vi "Configure Reporting Dialog.vi"(8 "error in (no error)":errorcluster, 11 "Execution UI In":refnum<class "Execution UI.lvclass">) -> (0 "error out":errorcluster, 2 "Reporting Enabled?":bool, 3 "Execution UI Out":refnum<class "Execution UI.lvclass">)   [LabVIEW 2020, in "Execution UI.lvclass"]
uses:
  Execution UI.lvclass
  Framework/Report Plugin/Report Plugin.lvclass
  Framework/Plugin Loader/Plugin Loader.lvlib
  Configuration Manager/UI Configuration Manager.lvclass
  Framework/Configuration Manager/Configuration Manager.lvclass
  Framework/Plugin/Plugin.lvclass
panel:
  in  "Reports Plugins":i32(listbox)
  in  "Configure":bool
  in  "Commit":bool
  in  "Cancel":bool
  # "Double Click to toggle active plugin"
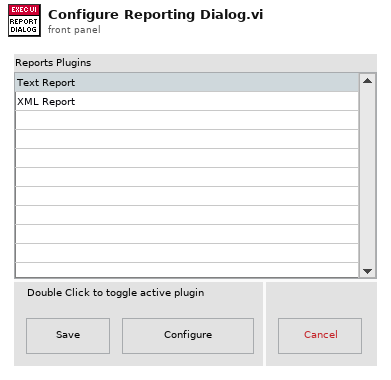
[diagram p1: front panel]
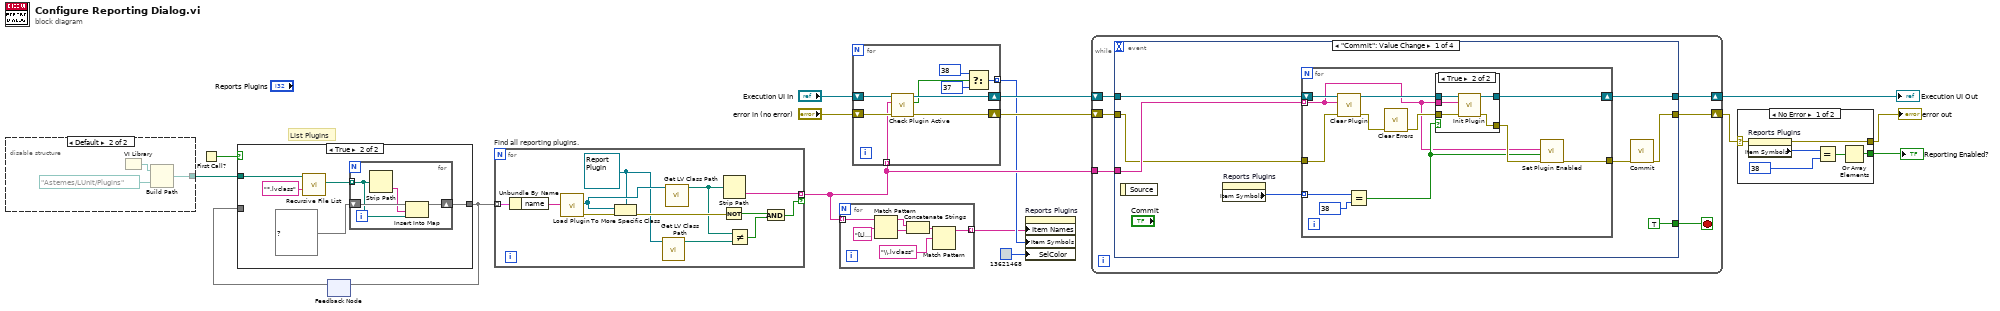
[diagram p0: block diagram]
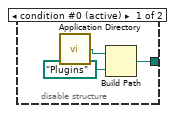
[diagram p2: hidden frame]
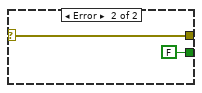
[diagram p4: hidden frame]
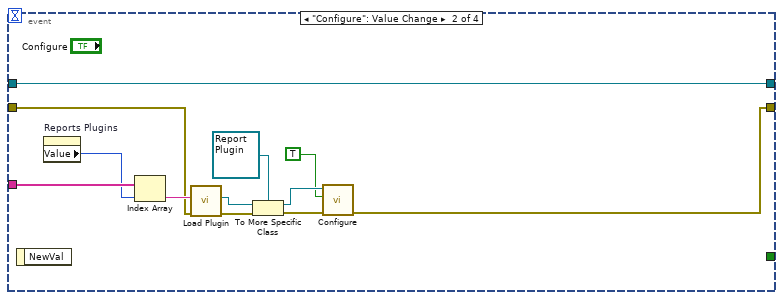
[diagram p6: hidden frame]
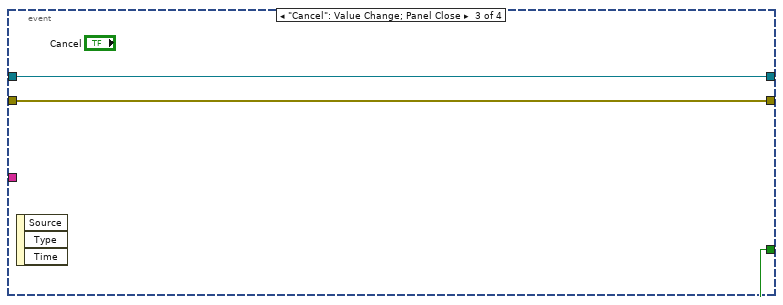
[diagram p7: hidden frame]
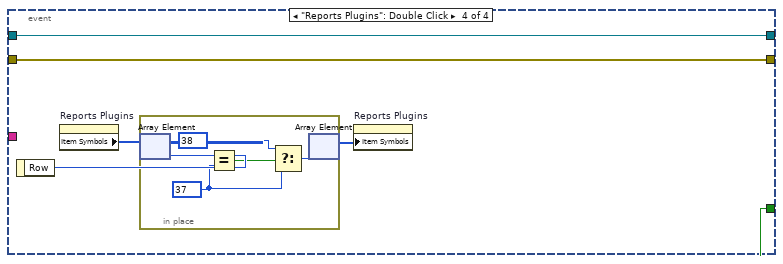
[diagram p8: hidden frame]
diagram:
  # "List Plugins"
  n1 = disable-structure shown="Default" {
    disable-tunnel: [w17 w20] -> w5
    frame condition #0 (active) {
      n2 = call <vilib>:"Application Directory.vi"() -> ("Application Directory"=w19:path)
      n3 = Build Path(base path=w19, name or relative path=path "Plugins") -> (appended path=w17:path)
    }
    frame condition #1 {
      n4 = VI Library() -> (path=w22:path)
      n5 = Build Path(base path=w22, name or relative path=path "Astemes/LUnit/Plugins") -> (appended path=w20:path)
    }
  }
  n6 = First Call?() -> (First Call?: T/F=w8:bool)
  n7 = feedback #1() -> (w9:map{string, path})  [unwired: 1 in]
  n8 = case shown="True" w8 {
    tunnel: w5 -> [_ w25]
    tunnel: [w23 w24] -> w10
    tunnel: w9 -> [w23 _]
    frame False {
    }
    frame True {
      n9 = call <vilib>:"Recursive File List.vi"("pattern"="*.lvclass", "Folder Path"=w25) -> ("All Files in Dir"=w26:path[])  [unwired: 5 in, 4 out]
      n10 = for {
        shift-right: [w31] -> w24
        shift-left: map{string, path} {} ("map") -> [w32]
        tunnel: w26 -> [w29] mode=indexing
        n11 = Strip Path(path=w29) -> (name=w30:string)  [unwired: 1 out]
        n12 = Insert Into Map(map in=w32, key=w30, value=w29) -> (map out=w31:map{string, path})  [unwired: 2 out]
      }
    }
  }
  n13 = feedback-in #1(w10) -> ()
  n14 = for "Find all reporting plugins." {
    tunnel: w10 -> [w44] mode=indexing
    tunnel: [w39] -> w11 mode=indexing if=w38
    w35 = refnum<class "Report Plugin.lvclass"> refnum ("Reports.lvlib:Report Interface.lvclass")
    n15 = Unbundle By Name(w44) -> ("name"=w33:string)
    n16 = call "Load Plugin.vi"("Plugin"=w33) -> ("error out"=w43:errorcluster, "Plugin"=w42:refnum<class "Plugin.lvclass">)  [unwired: 9 in]
    n17 = To More Specific Class(target class=w35, reference=w42, error in=w43) -> (error out=w41:errorcluster)  [unwired: 1 out]
    n18 = call <vilib>:"Get LV Class Path.vi"("object"=w35) -> ("class path"=w37:path)  [unwired: 9 in, 1 out]
    n19 = call <vilib>:"Get LV Class Path.vi"("object"=w42) -> ("class path"=w34:path)  [unwired: 9 in, 1 out]
    n20 = Not(x=w41) -> (.not. x?=w40:bool)
    n21 = Strip Path(path=w34) -> (name=w39:string)  [unwired: 1 out]
    n22 = Not Equal?(x=w34, y=w37) -> (x != y?=w36:bool)
    n23 = Compound Arithmetic op=AND(w40, w36) -> (w38:bool)
  }
  n24 = for {
    tunnel: w11 -> [w50] mode=indexing
    tunnel: [w47] -> w6 mode=indexing
    n25 = Match Pattern(string=w50, regular expression="[Ll][Uu][Nn][Ii][Tt] ") -> (before substring=w45:string, after substring=w49:string)  [unwired: 1 in, 2 out]
    n26 = Concatenate Strings(w45, w49) -> (w46:string)
    n27 = Match Pattern(string=w46, regular expression="\\.lvclass") -> (before substring=w47:string)  [unwired: 1 in, 3 out]
  }
  n28 = for {
    shift-right: [w59] -> w14
    shift-left: "Execution UI In" -> [w60]
    shift-right: [w57] -> w12
    shift-left: "error in (no error)" -> [w58]
    tunnel: w11 -> [w56] mode=indexing
    tunnel: [w52] -> w7 mode=indexing
    n29 = call "Check Plugin Active.vi"("error in (no error)"=w58, "Plugin"=w56, "Execution UI in"=w60) -> ("error out"=w57:errorcluster, "Active?"=w53:bool, "Execution UI out"=w59:refnum<class "Execution UI.lvclass">)  [unwired: 6 in]
    n30 = Select(t=38, s=w53, f=37) -> (s? t:f=w52:i32)
  }
  n31 = property on="Reports Plugins" class="LstBox (strict)"("Item Names"=w6, "Item Symbols"=w7, "SelColor"=u32 13621468 ("Primary Light")) -> ()  [unwired: 2 in, 2 out]
  n32 = while {
    tunnel: w11 -> [w62]
    shift-right: [w66] -> w16
    shift-left: w14 -> [w64]
    shift-right: [w65] -> w3
    shift-left: w12 -> [w63]
    stop <- w61 stop-if-true
    n33 = event shown="[0] \"Commit\": Value Change" {
      selector: _ -> [_ _ _ _]
      dyn-events: _ -> [_ _ _ _]
      timeout: _ -> [_ _ _ _]
      tunnel: [w73 w95 w107 w111] -> w66
      tunnel: w64 -> [w74 w95 w107 w111]
      tunnel: w63 -> [w69 w94 w108 w110]
      tunnel: [w67 w97 w108 w110] -> w65
      tunnel: w62 -> [w72 w105 _ _]
      tunnel: [TRUE _ TRUE FALSE] -> w61
      event "Commit": Value Change {
        n34 = event-data() -> ()  [unwired: 1 in, 1 out]
        n35 = property on="Reports Plugins" class="LstBox (strict)"() -> ("Item Symbols"=w70:i32[])  [unwired: 2 in, 2 out]
        n36 = for {
          tunnel: w72 -> [w75] mode=indexing
          tunnel: [w77] -> w68
          shift-right: [w83] -> w73
          shift-left: w74 -> [w86]
          tunnel: w70 -> [w81] mode=indexing
          tunnel: w69 -> [w79]
          n37 = call "Clear Plugin.vi"("error in (no error)"=w79, "Plugin"=w75, "Execution UI in"=w86) -> ("error out"=w82:errorcluster, "Execution UI out"=w84:refnum<class "Execution UI.lvclass">)  [unwired: 7 in]
          n38 = Equal?(x=w81, y=38) -> (x = y?=w76:bool)
          n39 = call <vilib>:"Clear Errors.vi"("error in (no error)"=w82) -> ("error out"=w85:errorcluster)  [unwired: 5 in, 1 out]
          n40 = case shown="True" w76 {
            tunnel: w85 -> [w88 w93]
            tunnel: w84 -> [w87 w92]
            tunnel: [w87 w91] -> w83
            tunnel: [w88 w89] -> w78
            tunnel: w75 -> [_ w90]
            frame False {
            }
            frame True {
              n41 = call "Init Plugin.vi"("error in (no error)"=w93, "Plugin"=w90, "Execution UI in"=w92) -> ("error out"=w89:errorcluster, "Execution UI out"=w91:refnum<class "Execution UI.lvclass">)  [unwired: 7 in]
            }
          }
          n42 = call "Set Plugin Enabled.vi"("error in (no error)"=w78, "Enabled?"=w76, "Plugin"=w75) -> ("error out"=w77:errorcluster)  [unwired: 8 in]
        }
        n43 = call "Commit.vi"("error in (no error)"=w68) -> ("error out"=w67:errorcluster)  [unwired: 10 in]
      }
      event "Configure": Value Change {
        n44 = event-data() -> ()  [unwired: 1 in, 1 out]
        n45 = property on="Reports Plugins" class="LstBox (strict)"() -> ("Value"=w104:i32)  [unwired: 2 in, 2 out]
        n46 = Index Array(array=w105, index=w104) -> (element=w103:string)
        n47 = call "Load Plugin.vi"("error in (no error)"=w94, "Plugin"=w103) -> ("error out"=w100:errorcluster, "Plugin"=w101:refnum<class "Plugin.lvclass">)  [unwired: 8 in]
        n48 = To More Specific Class(target class=refnum<class "Report Plugin.lvclass"> refnum ("Reports.lvlib:Report Interface.lvclass"), reference=w101, error in=w100) -> (specific class reference=w99:refnum<class "Report Plugin.lvclass">, error out=w98:errorcluster)
        n49 = call-dynamic "Configure.vi"("error in (no error)"=w98, "Interactive?"=TRUE, "Report Interface in"=w99) -> ("error out"=w97:errorcluster)  [unwired: 7 in, 1 out]
      }
      event "Cancel": Value Change; Panel Close {
        n50 = event-data() -> ()  [unwired: 1 in, 3 out]
      }
      event "Reports Plugins": Double Click {
        n51 = event-data() -> ("Row"=w113:i32)  [unwired: 1 in]
        n52 = property on="Reports Plugins" class="LstBox (strict)"() -> ("Item Symbols"=w114:i32[])  [unwired: 2 in, 2 out]
        n53 = in-place {
          w117 = 37
          n54 = in-place-array #2(w114, w113) -> (w119:i32)
          n55 = Equal?(x=w119, y=w117) -> (x = y?=w116:bool)
          n56 = Select(t=38, s=w116, f=w117) -> (s? t:f=w115:i32)
          n57 = in-place-array #2(w115) -> (w112:i32[])  [unwired: 1 out]
        }
        n58 = property on="Reports Plugins" class="LstBox (strict)"("Item Symbols"=w112) -> ()  [unwired: 2 in, 2 out]
      }
    }
  }
  "Execution UI Out" <- w16
  n59 = case shown="No Error" w3 {
    selector: w3 -> [w121 w127]
    tunnel: [w122 FALSE] -> w2
    tunnel: [w120 w127] -> w1
    frame No Error {
      n60 = property on="Reports Plugins" class="LstBox (strict)"(error in=w121) -> (error out=w120:errorcluster, "Item Symbols"=w125:i32[])  [unwired: 1 in, 1 out]
      n61 = Equal?(x=w125, y=38) -> (x = y?=w123:bool[])
      n62 = Or Array Elements(Boolean array=w123) -> (logical OR=w122:bool)
    }
    frame Error {
    }
  }
  "error out" <- w1
  "Reporting Enabled?" <- w2
